vi "PID_eventos.vi"() -> ()   [LabVIEW 2015]
uses:
  <vilib>/Instr/_visa.llb/VISA Configure Serial Port (Instr).vi
panel:
  out "Waveform Chart":dynamicdata(graph)
  in  "stop":bool
  out "read buffer":string
  in  "PUERTO":refnum<visa-resource-name>="COM4"
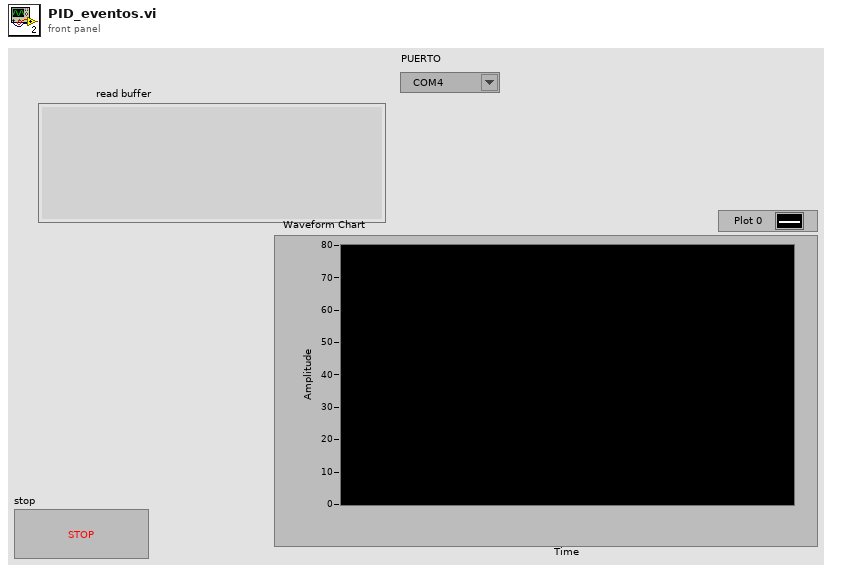
[diagram p1: front panel]
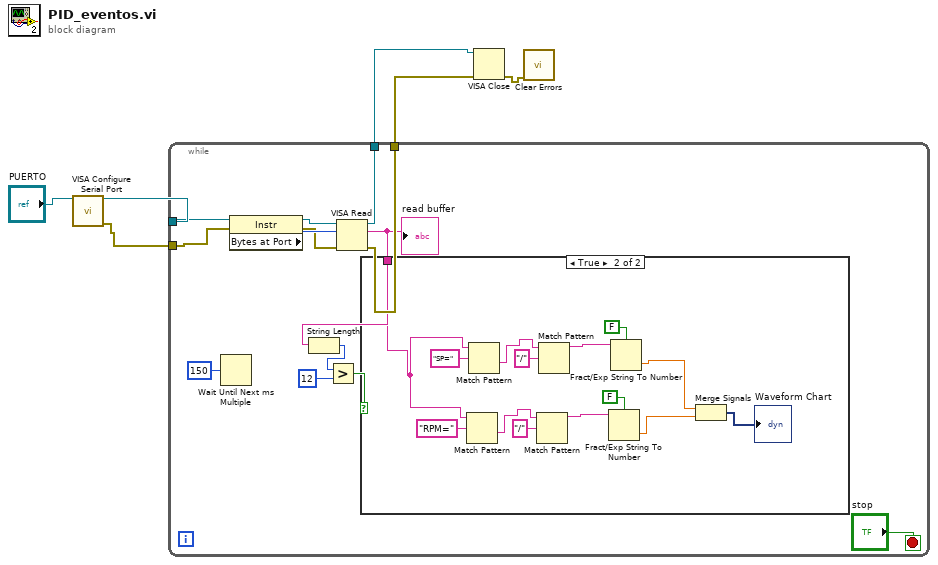
[diagram p0: block diagram]
diagram:
  n1 = call-poly "VISA Configure Serial Port"("VISA resource name"="PUERTO") -> ("VISA resource name out"=w3:refnum<visa-resource-name>, "error out"=w4:errorcluster)  [unwired: 13 in]
  n2 = while {
    tunnel: w4 -> [w15]
    tunnel: w3 -> [w16]
    tunnel: [w12] -> w2
    tunnel: [w11] -> w1
    stop <- "stop" stop-if-true
    n3 = Wait Until Next ms Multiple(millisecond multiple=u32 150) -> ()  [unwired: 1 out]
    n4 = property class="Instr"(reference=w16, error in=w15) -> (reference out=w18:refnum<visa-resource-name>, error out=w17:errorcluster, "Bytes at Port"=w19:u32)
    n5 = VISA Read(VISA resource name=w18, byte count=w19, error in (no error)=w17) -> (VISA resource name out=w12:refnum<visa-resource-name>, read buffer=w10:string, error out=w11:errorcluster)  [unwired: 1 out]
    "read buffer" <- w10
    n6 = String Length(string=w10) -> (length=w9:i32)
    n7 = Greater?(x=w9, y=12) -> (0:w7:bool)
    n8 = case shown="True" w7 {
      tunnel: w10 -> [_ w21]
      frame False {
      }
      frame True {
        n9 = Match Pattern(string=w21, regular expression="RPM=") -> (after substring=w27:string)  [unwired: 1 in, 3 out]
        n10 = Match Pattern(string=w21, regular expression="SP=") -> (after substring=w30:string)  [unwired: 1 in, 3 out]
        n11 = Match Pattern(string=w27, regular expression="/") -> (before substring=w28:string)  [unwired: 1 in, 3 out]
        n12 = Match Pattern(string=w30, regular expression="/") -> (before substring=w29:string)  [unwired: 1 in, 3 out]
        n13 = Fract/Exp String To Number(use system decimal point (T)=FALSE, string=w28) -> (number=w22:dbl)  [unwired: 2 in, 1 out]
        n14 = Fract/Exp String To Number(use system decimal point (T)=FALSE, string=w29) -> (number=w23:dbl)  [unwired: 2 in, 1 out]
        n15 = Merge Signals(w23, w22) -> (→"Waveform Chart":dynamicdata)
      }
    }
  }
  n16 = VISA Close(VISA resource name=w2, error in (no error)=w1) -> (error out=w5:errorcluster)
  n17 = call <vilib>:"Clear Errors.vi"("error in (no error)"=w5) -> ()  [unwired: 5 in, 2 out]
